vi "Construct PLC.vi"(6 "MB Data Block (default)":refnum<class "MB Data Block.lvclass">, 7 "TCP Config":T1={"IP Address"="", "Port"=0, "Slave ID"=-1, "Timeout"=10000} {"Slave ID" format="%.0x"}, 8 "error in (no error)":errorcluster, 9 "PLC Config":T3={"Use TCP"=FALSE, "Reference Format"=6, "Swap Words"=FALSE, "Poll List"=[]} {"Reference Format" items=["4 Digits"=4, "5 Digits"=5, "6 Digits"=6]}, 10 "Serial Config":T2={"COM Port"="COM1", "Slave ID"=1, "baud rate (bps)"=460800, "Mode"=enum."RTU", "Parity"=0, "Flow Control"=0, "Timeout"=200, "Retries"=1, "Stop Bits"=10} {"Stop Bits" items=["1.0"=10, "1.5"=15, "2.0"=20]; "Flow Control" items=["None", "XON/XOFF", "RTS/CTS", "XON/XOFF & RTS/CTS", "DTR/DSR", "XON/XOFF & DTR/DSR"]; "Parity" items=["None", "Odd", "Even", "Mark", "Space"]}, 11 "PLC in":refnum<class "MB PLC Client.lvclass">) -> (0 "error out":errorcluster, 3 "PLC out":refnum<class "MB PLC Client.lvclass">)   [LabVIEW 2018, in "MB PLC Client.lvlib" / "MB PLC Client.lvclass"]
uses:
  MB PLC Client.lvclass
  Types/PLC Config_Cluster.ctl
  Types/MB Ref Range_Cluster.ctl
  Types/Serial Config_Cluster.ctl
  Types/TCP Config_Cluster.ctl
  Data/MB Data Block.lvclass
  Data/MB Data Block.lvclass/MB Data Block.ctl
  MB PLC Client.lvclass/MB PLC Client.ctl
  Data/Read Initialized.vi
  MB PLC Client.lvlib
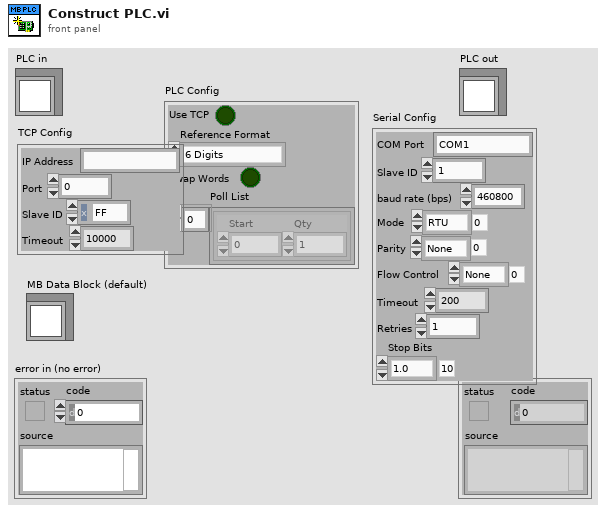
[diagram p1: front panel]
types:
  T1 = typedef "MB PLC Client.lvlib/TCP Config_Cluster.ctl" = cluster{"IP Address":string, "Port":u16, "Slave ID":i8, "Timeout":i32}
  T2 = typedef "MB PLC Client.lvlib/Serial Config_Cluster.ctl" = cluster{"COM Port":string, "Slave ID":u8, "baud rate (bps)":u32, "Mode":enum16{"RTU", "ASCII"}, "Parity":u16, "Flow Control":u16, "Timeout":u32, "Retries":u8, "Stop Bits":u16}
  T3 = typedef "MB PLC Client.lvlib/PLC Config_Cluster.ctl" = cluster{"Use TCP":bool, "Reference Format":u16, "Swap Words":bool, "Poll List":T4[]}
  T4 = typedef "MB PLC Client.lvlib/MB Ref Range_Cluster.ctl" = cluster{"Start":u32, "Qty":u16}
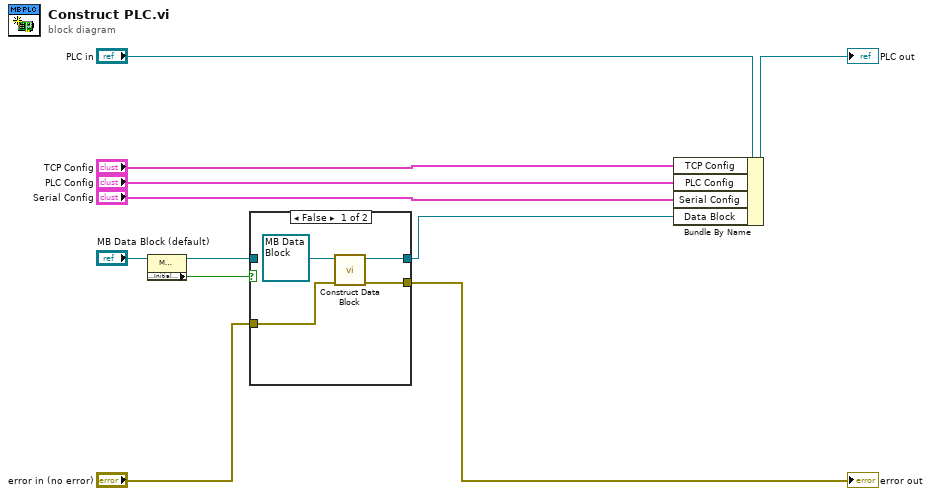
[diagram p0: block diagram]
diagram:
  n1 = property class="MB Data Block"(reference="MB Data Block (default)") -> (reference out=w1:refnum<class "MB Data Block.lvclass">, "Properties:Initialized"=w2:bool)  [unwired: 1 in, 1 out]
  n2 = case shown="False" w2 {
    tunnel: w1 -> [_ w17]
    tunnel: [w14 w17] -> w4
    tunnel: "error in (no error)" -> [w13 w16]
    tunnel: [w12 w16] -> w5
    frame False {
      n3 = call-dynamic "Construct Data Block.vi"("error in (no error)"=w13, "Modbus Data Store in"=refnum<class "MB Data Block.lvclass"> refnum) -> ("error out"=w12:errorcluster, "Modbus Data Store out"=w14:refnum<class "MB Data Block.lvclass">)  [unwired: 8 in]
    }
    frame True {
    }
  }
  "error out" <- w5
  n4 = Bundle By Name(cluster="PLC in", "TCP Config"="TCP Config", "PLC Config"="PLC Config", "Serial Config"="Serial Config", "Data Block"=w4) -> (→"PLC out":refnum<class "MB PLC Client.lvclass">)
